vi "测试.vi"() -> ()   [LabVIEW 2020]
uses:
  8649b9f9-8ffd-41c6-913b-8276f7b27aa5.vi
  viLib/LogLib/LogLib.lvlib
  viLib/QueueLib/QueueLib.lvlib
  6d43c680-a1f8-4723-bf79-b62a09ce1ae1.vi
  Lib/2601B/2601B.lvclass
  D:/Workspace/LabVIEW/MemristorCharacterization/Lib/2601B/2601B.lvclass
panel:
  out "触发按钮":T1(tab)
  in  "扫描负":bool
  in  "扫描正":bool
  in  "循环":bool
  out "剩余":u32
  in  "次数":u32=1 min=1 max=100
  in  "保持时间":bool
  in  "脉冲2":bool
  in  "脉冲1":bool
  in  "高速脉冲1":bool
  in  "高速脉冲2":bool
  in  "任意波形":bool
  in  "功能选择":T2(xcontrol)
  in  "样品标记":string(combo)
  in  "停止":bool
  in  "数据显示":dbl[][](xcontrol)
  out "测试人员":string
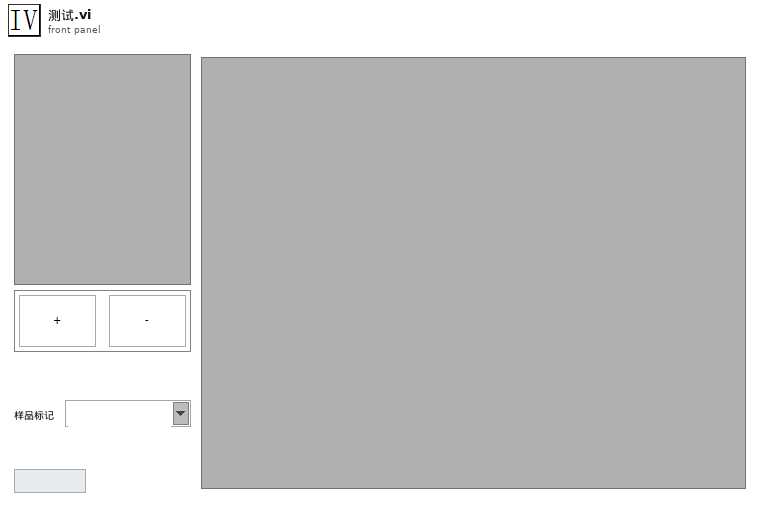
[diagram p1: front panel]
types:
  T1 = enum32{"扫描", "循环扫描", "保持时间", "脉冲", "高速脉冲", "任意波形"}
  T2 = enum16{"扫描", "循环扫描", "保持时间", "脉冲", "高速脉冲", "任意波形"}
  T3 = typedef "队列组.ctl" = cluster{"2601B":refnum<queue>, "数据处理":refnum<queue>}
  T4 = typedef "功能选择.xctl/方向属性.ctl" = enum16{"1", "2"}
  T5 = enum8{"Enabled", "Disabled", "Disabled and Grayed Out"}
  T6 = typedef "QueueLib.lvlib/数据类型.ctl" = cluster{"消息":string, "数据":variant}
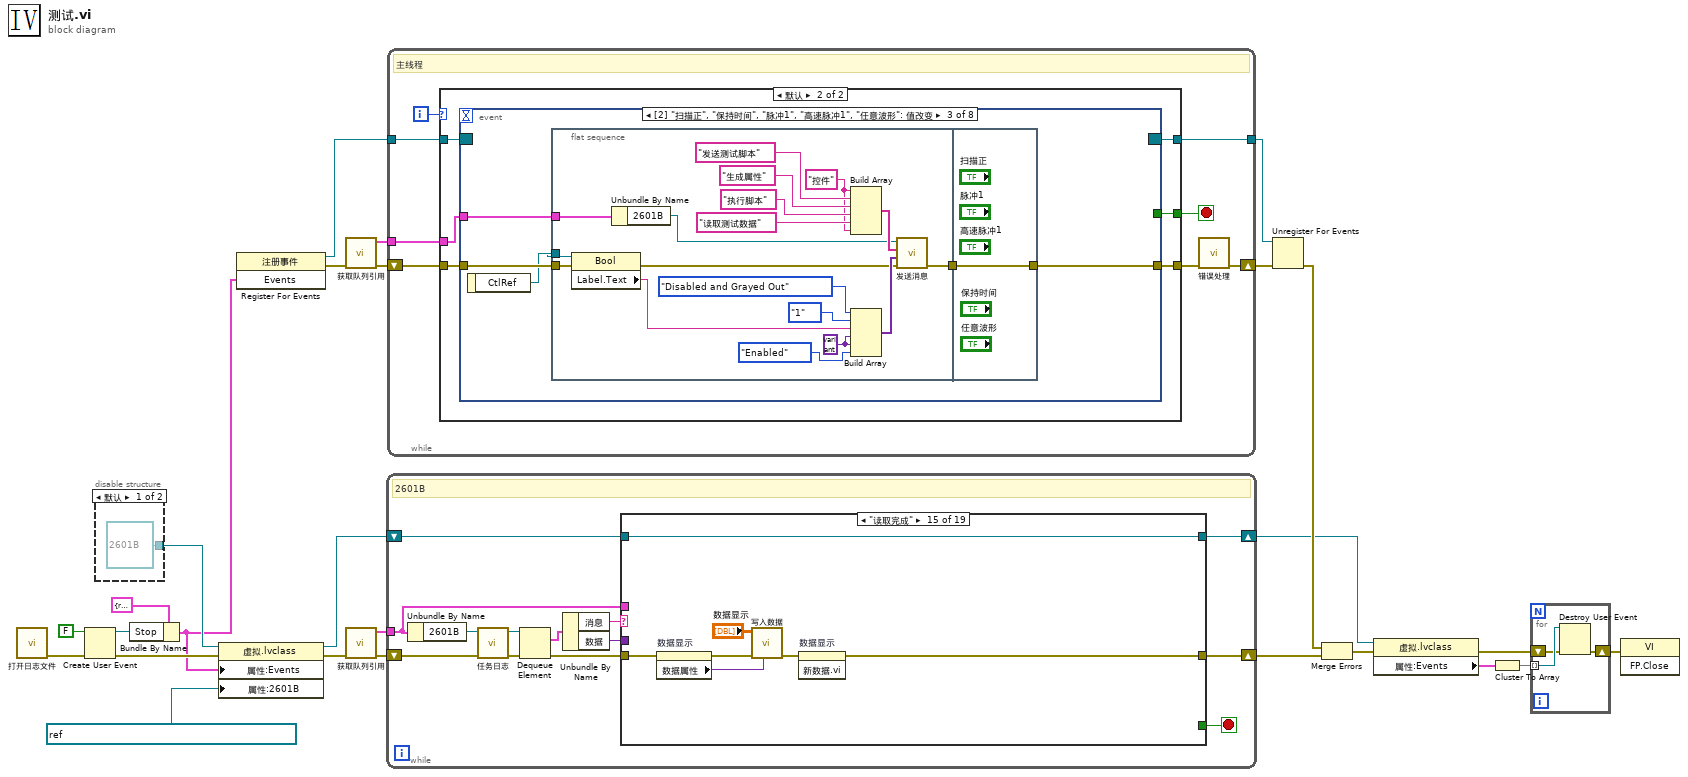
[diagram p0: block diagram]
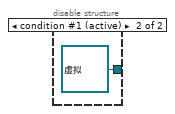
[diagram p2: hidden frame]
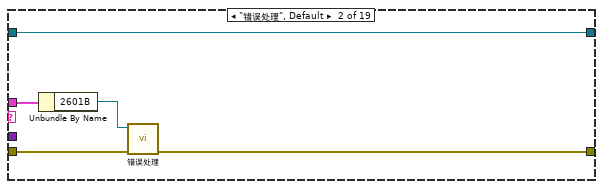
[diagram p4: hidden frame]
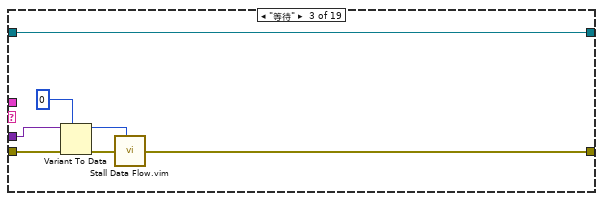
[diagram p5: hidden frame]
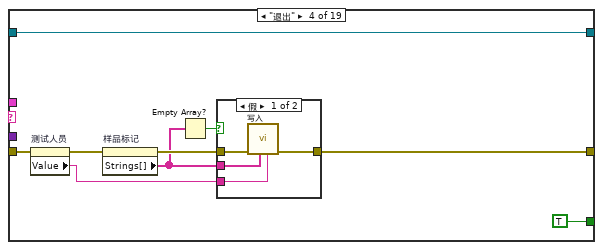
[diagram p6: hidden frame]
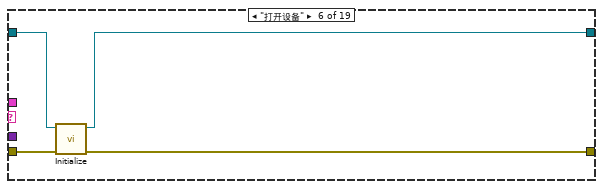
[diagram p9: hidden frame]
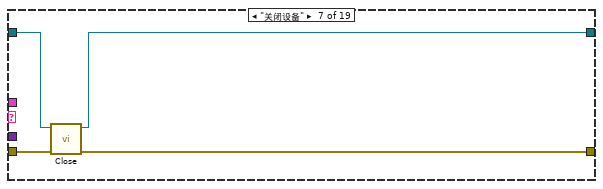
[diagram p10: hidden frame]
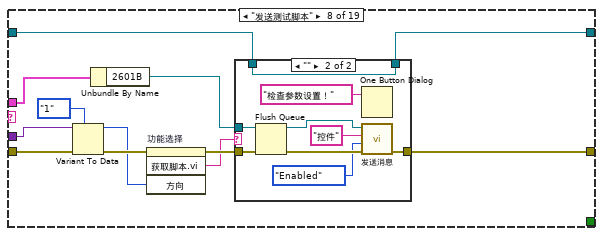
[diagram p11: hidden frame]
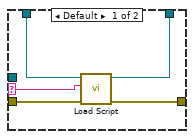
[diagram p12: hidden frame]
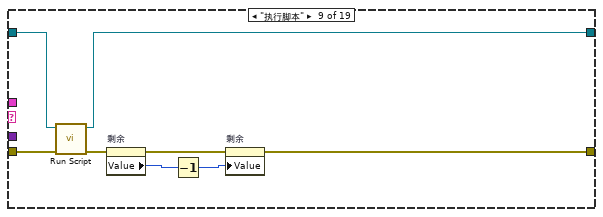
[diagram p13: hidden frame]
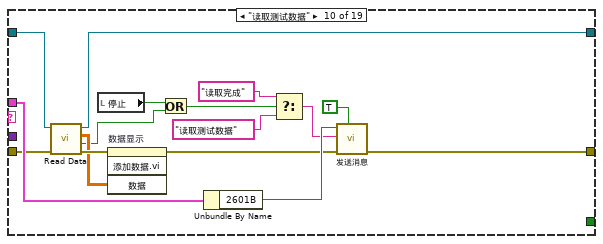
[diagram p14: hidden frame]
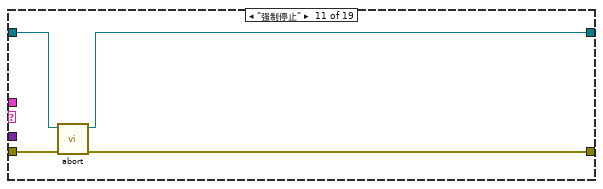
[diagram p15: hidden frame]
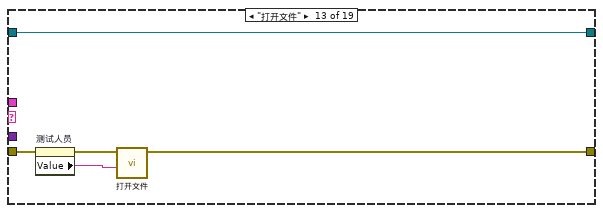
[diagram p17: hidden frame]
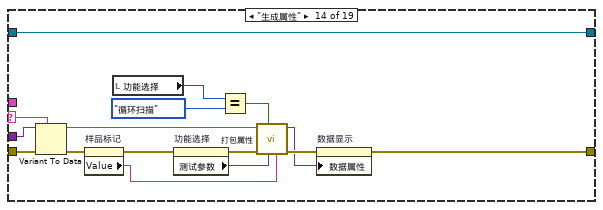
[diagram p18: hidden frame]
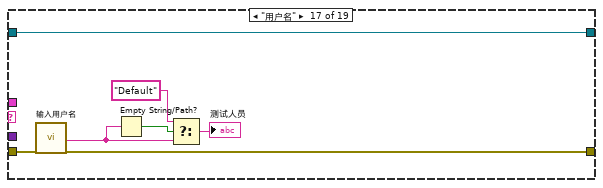
[diagram p20: hidden frame]
diagram:
  n1 = call "打开日志文件.vi"() -> ("错误输出"=w2:errorcluster)  [unwired: 11 in]
  n2 = Create User Event(user event datatype=FALSE ("事件数据"), error in=w2) -> (user event=w19:refnum<user-event>, error out=w15:errorcluster)
  n3 = disable-structure shown="默认" {
    disable-tunnel: [refnum<class "2601B.lvclass"> refnum ("2601B.lvclass") refnum<class "虚拟.lvclass"> refnum ("虚拟.lvclass")] -> w22
    frame condition #0 {
    }
    frame condition #1 (active) {
    }
  }
  n4 = Bundle By Name(cluster=cluster{"Stop":refnum<user-event>} {"Stop"=refnum} ("Events"), "Stop"=w19) -> (w14:cluster{"Stop":refnum<user-event>})
  n5 = property class="虚拟.lvclass"(reference=w22, error in=w15, "属性:Events"=w14, "属性:2601B"=refnum<visa-resource-name> "USB0::0x05E6::0x2601::4469244::INSTR" ("2601B")) -> (reference out=w16:refnum<class "虚拟.lvclass">, error out=w17:errorcluster)
  n6 = register-events(w14) -> (reference out=w13:refnum<event-registration>, error out=w1:errorcluster)  [unwired: 2 in]
  n7 = call "获取队列引用.vi"("错误输入（无错误）"=w1) -> ("错误输出"=w25:errorcluster, "队列组"=w26:T3)  [unwired: 9 in]
  n8 = call "获取队列引用.vi"("错误输入（无错误）"=w17) -> ("错误输出"=w23:errorcluster, "队列组"=w24:T3)  [unwired: 9 in]
  n9 = while {
    tunnel: w24 -> [w36]
    shift-right: [w37] -> w10
    shift-left: w23 -> [w35]
    shift-right: [w29] -> w7
    shift-left: w16 -> [w30]
    stop <- w31 stop-if-true
    # "2601B"
    n10 = Unbundle By Name(w36) -> ("2601B"=w33:refnum<queue>)
    n11 = call "任务日志.vi"("错误输入（无错误）"=w35, "队列输入"=w33) -> ("错误输出"=w34:errorcluster, "队列输出"=w32:refnum<queue>)  [unwired: 8 in]
    n12 = Dequeue Element(queue=w32, error in (no error)=w34) -> (element=w41:T6, error out=w40:errorcluster)  [unwired: 1 in, 2 out]
    n13 = Unbundle By Name(w41) -> ("消息"=w39:string, "数据"=w38:variant)
    n14 = case shown="\"读取完成\"" w39 {
      selector: w39 -> [_ _ _ _ _ _ _ _ _ _ _ _ _ w153 _ _ _ _ _]
      tunnel: [w43 w47 w52 w56 w71 w75 w78 w82 w110 w124 w132 w135 w136 w143 w159 w165 w171 w177 w192] -> w37
      tunnel: w40 -> [w43 w48 w55 w61 w71 w74 w79 w90 w108 w128 w133 w135 w137 w156 w160 w165 w170 w178 w191]
      tunnel: w38 -> [_ _ w53 _ _ _ _ w91 _ _ _ _ _ w154 _ _ _ _ w189]
      tunnel: w36 -> [_ w46 _ _ _ _ _ w85 _ w129 _ _ _ _ _ _ _ _ _]
      tunnel: [_ _ _ TRUE ("事件数据") _ _ _ _ _ _ _ _ _ _ _ _ _ _ _] -> w31
      tunnel: w30 -> [w42 w44 w49 w60 w70 w73 w76 w81 w107 w126 w130 w134 w140 w145 w163 w164 w172 w179 w182]
      tunnel: [w42 w44 w49 w60 w70 w72 w77 w80 w106 w127 w131 w134 w140 w145 w163 w164 w172 w179 w182] -> w29
      frame "==== 标准任务 ====" {
      }
      frame "错误处理", Default {
        n15 = Unbundle By Name(w46) -> ("2601B"=w45:refnum<queue>)
        n16 = call "错误处理.vi"("错误输入（无错误）"=w48, "队列输入"=w45) -> ("错误输出"=w47:errorcluster)  [unwired: 8 in, 1 out]
      }
      frame "等待" {
        n17 = Variant To Data(error in=w55, type=u32 0 ("milliseconds to wait"), Variant=w53) -> (data=w50:u32, error out=w54:errorcluster)
        n18 = call "Stall Data Flow.vim"("value in"=w54, "milliseconds to wait"=w50) -> ("value out"=w52:errorcluster)  [unwired: 1 out]
      }
      frame "退出" {
        n19 = property on="测试人员" class="Str"(error in=w61) -> (error out=w63:errorcluster, "Value"=w62:string)  [unwired: 1 in, 1 out]
        n20 = property on="样品标记" class="CmbBox"(error in=w63) -> (error out=w64:errorcluster, "Strings[]"=w57:string[])  [unwired: 1 in, 1 out]
        n21 = Empty Array?(array=w57) -> (empty?=w58:bool)
        n22 = case shown="假" w58 {
          tunnel: w64 -> [w68 w69]
          tunnel: [w67 w69] -> w56
          tunnel: w62 -> [w66 _]
          tunnel: w57 -> [w65 _]
          frame False {
            n23 = call "写入.vi"("测试人员"=w66, "样品标记"=w65, "error in (no error)"=w68) -> ("error out"=w67:errorcluster)  [unwired: 8 in]
          }
          frame True {
          }
        }
      }
      frame "==== 2601B ====" {
      }
      frame "打开设备" {
        n24 = call-dynamic "Initialize.vi"("error in (no error)"=w74, "虚拟 输入"=w73) -> ("error out"=w75:errorcluster, "虚拟 输出"=w72:refnum<class "虚拟.lvclass">)  [unwired: 8 in]
      }
      frame "关闭设备" {
        n25 = call-dynamic "Close.vi"("error in (no error)"=w79, "虚拟 输入"=w76) -> ("error out"=w78:errorcluster, "虚拟 输出"=w77:refnum<class "虚拟.lvclass">)  [unwired: 8 in]
      }
      frame "发送测试脚本" {
        n26 = Variant To Data(error in=w90, type=方向属性."1" ("方向"), Variant=w91) -> (data=w87:T4, error out=w88:errorcluster)
        n27 = Unbundle By Name(w85) -> ("2601B"=w84:refnum<queue>)
        n28 = invoke on="功能选择" class="功能选择 (严格)" method="获取脚本.vi"(error in=w88, "方向"=w87) -> (error out=w86:errorcluster, "获取脚本.vi"=w83:string)  [unwired: 2 in, 2 out]
        n29 = case shown="\"\"" w83 {
          selector: w83 -> [w92 _]
          tunnel: w86 -> [w96 w105]
          tunnel: w84 -> [_ w104]
          tunnel: [w95 w99] -> w82
          tunnel: w81 -> [w94 w97]
          tunnel: [w93 w97] -> w80
          frame Default {
            n30 = call-dynamic "Load Script.vi"("error in (no error)"=w96, "Script"=w92, "虚拟 输入"=w94) -> ("error out"=w95:errorcluster, "虚拟 输出"=w93:refnum<class "虚拟.lvclass">)  [unwired: 7 in]
          }
          frame "" {
            n31 = Flush Queue(queue=w104, error in (no error)=w105) -> (queue out=w102:refnum<queue>, error out=w103:errorcluster)  [unwired: 1 out]
            n32 = One Button Dialog(message="检查参数设置！" ("消息")) -> ()  [unwired: 1 in, 1 out]
            n33 = call-poly "发送消息.vi"("错误输入（无错误）"=w103, "数据"=T5."Enabled" ("禁用"), "消息"="控件", "输入队列"=w102) -> ("错误输出"=w99:errorcluster)  [unwired: 6 in, 1 out]
          }
        }
      }
      frame "执行脚本" {
        n34 = call-dynamic "Run Script.vi"("error in (no error)"=w108, "虚拟 输入"=w107) -> ("error out"=w109:errorcluster, "虚拟 输出"=w106:refnum<class "虚拟.lvclass">)  [unwired: 8 in]
        n35 = property on="剩余" class="DigNum (严格)"(error in=w109) -> (error out=w111:errorcluster, "Value"=w112:u32)  [unwired: 1 in, 1 out]
        n36 = Decrement(x=w112) -> (x-1=w113:u32)
        n37 = property on="剩余" class="DigNum (严格)"(error in=w111, "Value"=w113) -> (error out=w110:errorcluster)  [unwired: 1 in, 1 out]
      }
      frame "读取测试数据" {
        n38 = call-dynamic "Read Data.vi"("error in (no error)"=w128, "虚拟 输入"=w126) -> ("error out"=w122:errorcluster, "完成"=w115:bool, "DBL"=w117:dbl[][], "虚拟 输出"=w127:refnum<class "虚拟.lvclass">)  [unwired: 6 in]
        n39 = local read "停止"() -> (w116:bool)
        n40 = invoke on="数据显示" class="数据显示 (严格)" method="添加数据.vi"(error in=w122, "数据"=w117) -> (error out=w121:errorcluster)  [unwired: 2 in, 3 out]
        n41 = Or(x=w116, y=w115) -> (x .or. y?=w114:bool)
        n42 = Unbundle By Name(w129) -> ("2601B"=w125:refnum<queue>)
        n43 = Select(t="读取完成" ("消息"), s=w114, f="读取测试数据" ("消息")) -> (s? t:f=w118:string)
        n44 = call-poly "发送消息.vi"("强制优先"=TRUE, "错误输入（无错误）"=w121, "消息"=w118, "输入队列"=w125) -> ("错误输出"=w124:errorcluster)  [unwired: 6 in, 1 out]
      }
      frame "强制停止" {
        n45 = call-dynamic "abort.vi"("error in (no error)"=w133, "虚拟 输入"=w130) -> ("error out"=w132:errorcluster, "虚拟 输出"=w131:refnum<class "虚拟.lvclass">)  [unwired: 8 in]
      }
      frame "==== 数据 ====" {
      }
      frame "打开文件" {
        n46 = property on="测试人员" class="Str"(error in=w137) -> (error out=w139:errorcluster, "Value"=w138:string)  [unwired: 1 in, 1 out]
        n47 = call "打开文件.vi"("测试人员"=w138, "错误输入（无错误）"=w139) -> ("错误输出"=w136:errorcluster)  [unwired: 9 in]
      }
      frame "生成属性" {
        n48 = Variant To Data(error in=w156, type=w153, Variant=w154) -> (data=w149:string, error out=w155:errorcluster)
        n49 = property on="样品标记" class="CmbBox"(error in=w155) -> (error out=w151:errorcluster, "Value"=w152:string)  [unwired: 1 in, 1 out]
        n50 = local read "功能选择"() -> (w148:T2)
        n51 = property on="功能选择" class="功能选择 (严格)"(error in=w151) -> (error out=w150:errorcluster, "测试参数"=w142:variant)  [unwired: 1 in, 1 out]
        n52 = Equal?(x=w148, y=T2."循环扫描") -> (x = y?=w146:bool)
        n53 = call "打包属性.vi"("样品标记"=w152, "测试参数"=w142, "循环"=w146, "错误输入"=w150, "功能"=w149) -> ("错误输出"=w144:errorcluster, "数据属性"=w141:variant)  [unwired: 5 in]
        n54 = property on="数据显示" class="数据显示 (严格)"(error in=w144, "数据属性"=w141) -> (error out=w143:errorcluster)  [unwired: 1 in, 1 out]
      }
      frame "读取完成" {
        n55 = property on="数据显示" class="数据显示 (严格)"(error in=w160) -> (error out=w158:errorcluster, "数据属性"=w157:variant)  [unwired: 1 in, 1 out]
        n56 = call "写入数据.vi"("数据属性"=w157, "错误输入（无错误）"=w158, "测试数据"="数据显示") -> ("错误输出"=w161:errorcluster)  [unwired: 8 in]
        n57 = invoke on="数据显示" class="数据显示 (严格)" method="新数据.vi"(error in=w161) -> (error out=w159:errorcluster)  [unwired: 2 in, 2 out]
      }
      frame "==== 用户界面 ====" {
      }
      frame "用户名" {
        n58 = call "输入用户名"("error in (no error)"=w170) -> ("用户名"=w169:string, "error out"=w171:errorcluster)  [unwired: 16 in, 1 out]
        n59 = Empty String/Path?(string/path=w169) -> (empty?=w167:bool)
        n60 = Select(t="Default", s=w167, f=w169) -> (s? t:f=→"测试人员":string)
      }
      frame "读取样品标记" {
        n61 = property on="测试人员" class="Str"(error in=w178) -> (error out=w175:errorcluster, "Value"=w176:string)  [unwired: 1 in, 1 out]
        n62 = call "读取.vi"("测试人员"=w176, "error in (no error)"=w175) -> ("error out"=w174:errorcluster, "样品标记"=w173:string[])  [unwired: 8 in]
        n63 = property on="样品标记" class="CmbBox"(error in=w174, "Strings[]"=w173) -> (error out=w177:errorcluster)  [unwired: 1 in, 1 out]
      }
      frame "控件" {
        w183 = T5."Enabled" ("禁用")
        n64 = Variant To Data(error in=w191, type=w183, Variant=w189) -> (data=w184:T5, error out=w190:errorcluster)
        n65 = Not Equal?(x=w184, y=w183) -> (x != y?=w181:bool)
        n66 = property on="停止" class="Bool (严格)"(error in=w190, "Visible"=w181, "Value"=FALSE ("停止")) -> (error out=w186:errorcluster)  [unwired: 1 in, 1 out]
        n67 = property on="剩余" class="DigNum (严格)"(error in=w186, "Visible"=w181) -> (error out=w180:errorcluster)  [unwired: 1 in, 1 out]
        n68 = control-ref of="本VI"() -> (w188:refnum<vi>)
        n69 = call "禁用控件.vi"("控件名称"=string[] ["功能选择", "触发按钮", "样品标记"], "本VI"=w188, "错误输入（无错误）"=w180, "禁用"=w184) -> ("错误输出"=w192:errorcluster)  [unwired: 7 in]
      }
    }
  }
  n70 = while {
    tunnel: w26 -> [w198]
    shift-right: [w195] -> w12
    shift-left: w25 -> [w199]
    tunnel: w13 -> [w194]
    tunnel: [w193] -> w11
    i -> [w200]
    stop <- w197 stop-if-true
    # "主线程"
    n71 = case shown="默认" w200 {
      tunnel: w199 -> [w203 w219]
      tunnel: [w202 w217] -> w196
      tunnel: w198 -> [w204 w218]
      tunnel: [_ w215] -> w197
      tunnel: w194 -> [w201 w216]
      tunnel: [w201 w214] -> w193
      frame 0 {
        n72 = flat-sequence {
          tunnel: w204 -> [w213]
          tunnel: w203 -> [w212]
          tunnel: [w207] -> w202
          frame #0 {
            n73 = Unbundle By Name(w213) -> ("2601B"=w211:refnum<queue>)
            n74 = call-poly "发送消息.vi"("错误输入（无错误）"=w212, "消息"="打开设备", "输入队列"=w211) -> ("错误输出"=w208:errorcluster)  [unwired: 7 in, 1 out]
            n75 = control-ref of="本VI"() -> (w209:refnum<vi>)
            n76 = call "禁用控件.vi"("控件名称"=string[] ["功能选择", "触发按钮", "样品标记", "数据显示", "测试人员"], "本VI"=w209, "错误输入（无错误）"=w208, "禁用"=T5."Disabled and Grayed Out") -> ("错误输出"=w207:errorcluster)  [unwired: 7 in]
          }
        }
      }
      frame Default {
        n77 = event shown="[2] \"扫描正\", \"保持时间\", \"脉冲1\", \"高速脉冲1\", \"任意波形\": 值改变" {
          selector: w216 -> [_ _ _ _ _ _ _ _]
          dyn-events: [_ _ _ _ _ _ _ _] -> w214
          timeout: _ -> [_ _ _ _ _ _ _ _]
          tunnel: w219 -> [w221 w243 w250 w274 w295 w305 w320 w347]
          tunnel: [w223 w242 w247 w273 w297 w306 w321 w346] -> w217
          tunnel: w218 -> [_ _ w248 w272 w296 w307 w322 w345]
          tunnel: [_ _ _ _ _ _ w319 w344] -> w215
          event "样品标记": Value Change {
            n78 = event-data() -> ("NewVal"=w220:string, "OldVal"=w222:string)  [unwired: 1 in]
            n79 = flat-sequence {
              tunnel: [w226] -> w223
              tunnel: w220 -> [w231]
              tunnel: w222 -> [w230]
              tunnel: w221 -> [w227]
              frame #0 {
                n80 = property on="样品标记" class="CmbBox"(error in=w227) -> (error out=w225:errorcluster, "Strings[]"=w229:string[])  [unwired: 1 in, 1 out]
                n81 = case shown="\"\"" w231 {
                  selector: w231 -> [w233 _]
                  tunnel: w230 -> [_ w238]
                  tunnel: w229 -> [w236 w241]
                  tunnel: [w234 w239] -> w228
                  tunnel: w225 -> [w232 w237]
                  tunnel: [w232 w237] -> w224
                  frame Default {
                    n82 = Build Array (concatenate)(w236, w233) -> (w235:string[])
                    n83 = call "Remove Duplicates From 1D Array.vim"("array"=w235) -> ("array with duplicates removed"=w234:string[])  [unwired: 10 in]
                  }
                  frame "" {
                    n84 = Search 1D Array(1D array=w241, element=w238) -> (index of element=w240:i32)  [unwired: 1 in]
                    n85 = Delete From Array(array=w241, index=w240) -> (array with subset deleted=w239:string[])  [unwired: 1 in, 1 out]
                  }
                }
                n86 = property on="样品标记" class="CmbBox"(error in=w224, "Strings[]"=w228) -> (error out=w226:errorcluster)  [unwired: 1 in, 1 out]
              }
            }
          }
          event "功能选择": Value Change {
            n87 = event-data() -> ()  [unwired: 1 in, 1 out]
            n88 = flat-sequence {
              tunnel: w243 -> [w246]
              tunnel: [w245] -> w242
              frame #0 {
                n89 = property on="数据显示" class="数据显示 (严格)"(error in=w246, "扫描"="功能选择") -> (error out=w245:errorcluster)  [unwired: 1 in, 1 out]
                "触发按钮" <- "功能选择"
              }
            }
          }
          event "扫描正", "保持时间", "脉冲1", "高速脉冲1", "任意波形": Value Change {
            n90 = event-data() -> ("CtlRef"=w249:refnum<vi>)  [unwired: 1 in]
            n91 = flat-sequence {
              tunnel: w249 -> [w269]
              tunnel: w250 -> [w268]
              tunnel: w248 -> [w255]
              tunnel: [w256] -> w251
              tunnel: [w270] -> w247
              tunnel: w251 -> [w270]
              frame #0 {
                w262 = variant
                w252 = "控件" ("消息")
                n92 = property class="Bool"(reference=w269, error in=w268) -> (error out=w257:errorcluster, "Label.Text"=w260:string)  [unwired: 1 out]
                n93 = Unbundle By Name(w255) -> ("2601B"=w254:refnum<queue>)
                n94 = Build Array(w252, "发送测试脚本" ("消息"), "生成属性" ("消息"), "执行脚本" ("消息"), "读取测试数据" ("消息"), w252) -> (w259:string[])
                n95 = Build Array(T5."Disabled and Grayed Out" ("禁用"), 方向属性."1" ("方向"), w260, w262, w262, T5."Enabled" ("禁用")) -> (w258:variant[])
                n96 = call-poly "发送消息.vi"("错误输入（无错误）"=w257, "数据列表"=w258, "消息列表"=w259, "输入队列"=w254) -> ("错误输出"=w256:errorcluster)  [unwired: 6 in, 1 out]
              }
              frame #1 {
              }
            }
          }
          event "扫描负", "脉冲2", "高速脉冲2": Value Change {
            n97 = event-data() -> ("CtlRef"=w275:refnum<vi>)  [unwired: 1 in]
            n98 = flat-sequence {
              tunnel: w275 -> [w293]
              tunnel: w274 -> [w292]
              tunnel: w272 -> [w279]
              tunnel: [w280] -> w271
              tunnel: [w294] -> w273
              tunnel: w271 -> [w294]
              frame #0 {
                w286 = variant
                w276 = "控件" ("消息")
                n99 = property class="Bool"(reference=w293, error in=w292) -> (error out=w281:errorcluster, "Label.Text"=w284:string)  [unwired: 1 out]
                n100 = Unbundle By Name(w279) -> ("2601B"=w278:refnum<queue>)
                n101 = Build Array(w276, "发送测试脚本" ("消息"), "生成属性" ("消息"), "执行脚本" ("消息"), "读取测试数据" ("消息"), w276) -> (w283:string[])
                n102 = Build Array(T5."Disabled and Grayed Out" ("禁用"), 方向属性."2" ("方向"), w284, w286, w286, T5."Enabled" ("禁用")) -> (w282:variant[])
                n103 = call-poly "发送消息.vi"("错误输入（无错误）"=w281, "数据列表"=w282, "消息列表"=w283, "输入队列"=w278) -> ("错误输出"=w280:errorcluster)  [unwired: 6 in, 1 out]
              }
              frame #1 {
              }
            }
          }
          event "循环": Value Change {
            n104 = event-data() -> ()  [unwired: 1 in, 1 out]
            n105 = flat-sequence {
              tunnel: [w301] -> w297
              tunnel: w296 -> [w300]
              tunnel: w295 -> [w298]
              frame #0 {
                n106 = Unbundle By Name(w300) -> ("2601B"=w302:refnum<queue>)
                n107 = call "生成任务队列.vi"("循环次数"="次数") -> ("任务数据"=w304:variant[], "任务名称"=w303:string[])  [unwired: 9 in]
                n108 = call-poly "发送消息.vi"("错误输入（无错误）"=w298, "数据列表"=w304, "消息列表"=w303, "输入队列"=w302) -> ("错误输出"=w301:errorcluster)  [unwired: 6 in, 1 out]
                "剩余" <- "次数"
              }
            }
          }
          event "停止": Value Change {
            n109 = event-data() -> ()  [unwired: 1 in, 1 out]
            n110 = flat-sequence {
              tunnel: w307 -> [w316]
              tunnel: [w315] -> w306
              tunnel: w305 -> [w313]
              frame #0 {
                n111 = Unbundle By Name(w316) -> ("2601B"=w317:refnum<queue>)
                n112 = Flush Queue(queue=w317, error in (no error)=w313) -> (queue out=w314:refnum<queue>, error out=w312:errorcluster)  [unwired: 1 out]
                n113 = Build Array(variant, T5."Enabled" ("禁用")) -> (w308:variant[])
                n114 = call-poly "发送消息.vi"("错误输入（无错误）"=w312, "数据列表"=w308, "消息列表"=string[] ["强制停止", "控件"], "输入队列"=w314) -> ("错误输出"=w315:errorcluster)  [unwired: 6 in, 1 out]
              }
            }
          }
          event Panel Close? {
            n115 = event-data() -> ()  [unwired: 1 in, 1 out]
            n116 = flat-sequence {
              tunnel: [w323] -> w319
              tunnel: w322 -> [w333]
              tunnel: [w332] -> w321
              tunnel: w320 -> [w331]
              frame #0 {
                n117 = property on="停止" class="Bool (严格)"(error in=w331) -> (error out=w330:errorcluster, "Visible"=w327:bool)  [unwired: 1 in, 1 out]
                n118 = Select(t="停止先啊", s=w327, f="退出？" ("消息")) -> (s? t:f=w326:string)
                n119 = Two Button Dialog(message=w326) -> (T button?=w329:bool)  [unwired: 2 in]
                n120 = Compound Arithmetic op=AND ("复合运算")(invert w327, w329) -> (w328:bool)
                n121 = case shown="真" w328 {
                  selector: w328 -> [w334 w336]
                  tunnel: w333 -> [_ w343]
                  tunnel: [w335 w341] -> w332
                  tunnel: w330 -> [w335 w340]
                  tunnel: [w334 w336] -> w323
                  frame False {
                  }
                  frame True {
                    n122 = Unbundle By Name(w343) -> ("2601B"=w342:refnum<queue>)
                    n123 = Build Array("关闭设备" ("元素"), "退出" ("消息")) -> (w338:string[])
                    n124 = call-poly "发送消息.vi"("错误输入（无错误）"=w340, "消息列表"=w338, "输入队列"=w342) -> ("错误输出"=w341:errorcluster)  [unwired: 7 in, 1 out]
                  }
                }
              }
            }
            n125 = event-data("Discard?"=TRUE ("放弃？")) -> ()  [unwired: 1 in, 1 out]
          }
          event User Event {
            n126 = event-data() -> ("布尔"=w344:bool)  [unwired: 1 in]
            n127 = case shown="假" w344 {
              tunnel: w347 -> [w359 w362]
              tunnel: [w348 w361] -> w346
              tunnel: w345 -> [w358 w360]
              frame False {
                n128 = Unbundle By Name(w358) -> ("2601B"=w357:refnum<queue>)
                n129 = Build Array("用户名", "读取样品标记" ("元素"), "打开文件" ("元素")) -> (w356:string[])
                n130 = call-poly "发送消息.vi"("错误输入（无错误）"=w359, "消息列表"=w356, "输入队列"=w357) -> ("错误输出"=w349:errorcluster)  [unwired: 7 in, 1 out]
                n131 = control-ref of="本VI"() -> (w352:refnum<vi>)
                n132 = call "禁用控件.vi"("控件名称"=string[] ["功能选择", "触发按钮", "样品标记", "数据显示", "测试人员"], "本VI"=w352, "错误输入（无错误）"=w349, "禁用"=T5."Enabled") -> ("错误输出"=w348:errorcluster)  [unwired: 7 in]
              }
              frame True {
                n133 = Unbundle By Name(w360) -> ("2601B"=w364:refnum<queue>)
                n134 = call-poly "发送消息.vi"("错误输入（无错误）"=w362, "消息"="退出", "输入队列"=w364) -> ("错误输出"=w361:errorcluster)  [unwired: 7 in, 1 out]
              }
            }
          }
        }
      }
    }
    n135 = call "错误处理.vi"("错误输入（无错误）"=w196) -> ("错误输出"=w195:errorcluster)  [unwired: 9 in, 1 out]
  }
  n136 = Unregister For Events(event registration refnum=w11, error in=w12) -> (error out=w9:errorcluster)
  n137 = Merge Errors(w9, w10) -> (w8:errorcluster)
  n138 = property class="虚拟.lvclass"(reference=w7, error in=w8) -> (error out=w4:errorcluster, "属性:Events"=w6:cluster{"Stop":refnum<user-event>})  [unwired: 1 out]
  n139 = Cluster To Array(cluster=w6) -> (array=w5:refnum<user-event>[])
  n140 = for {
    tunnel: w5 -> [w367] mode=indexing
    shift-right: [w365] -> w3
    shift-left: w4 -> [w366]
    n141 = Destroy User Event(user event=w367, error in=w366) -> (error out=w365:errorcluster)
  }
  n142 = invoke class="VI" method="FP.Close"(error in=w3) -> ()  [unwired: 2 in, 3 out]
